vi "Delete_User.vi"(8 "error in (no error)":errorcluster, 11 "Name":string) -> (0 "error out":errorcluster, 3 "Result":bool)   [LabVIEW 2021]
uses:
  <vilib>/regexp/Match Regular Expression.xnode
panel:
  out "concatenated string":string
  out "standard output":string
  out "standard error":string
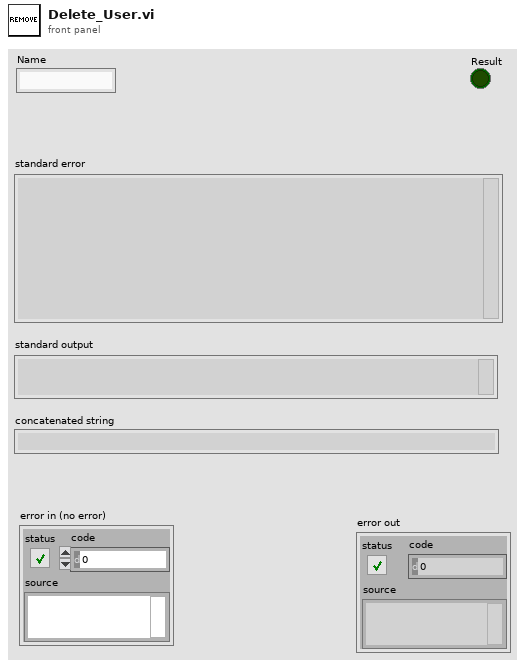
[diagram p1: front panel]
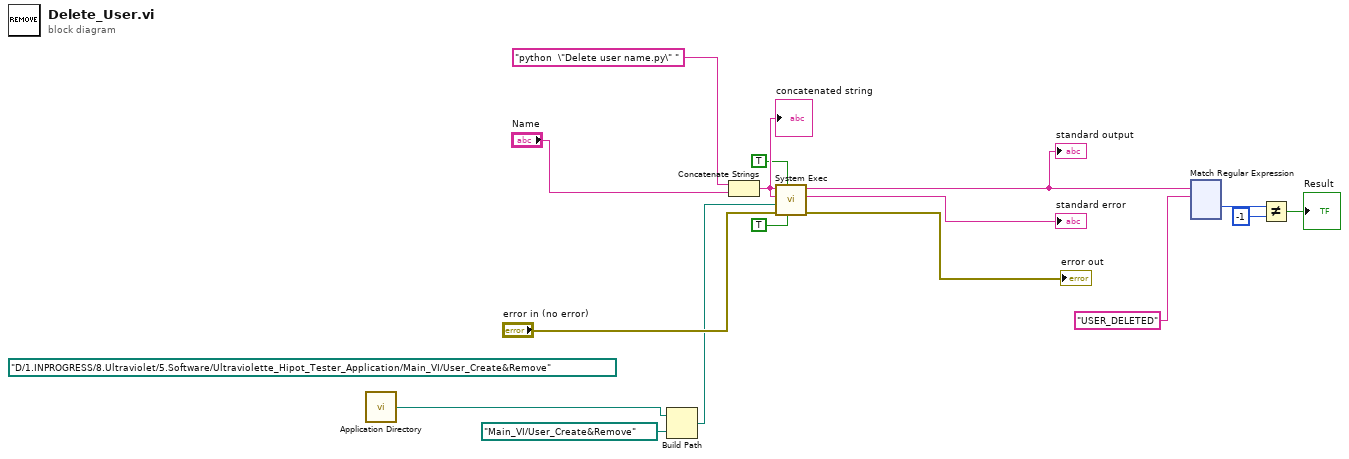
[diagram p0: block diagram]
diagram:
  (unwired) path "D:/1.INPROGRESS/8.Ultraviolet/5.Software/Ultraviolette_Hipot_Tester_Application/Main_VI/User_Create&Remove" ("working directory")
  n1 = call <vilib>:"Application Directory.vi"() -> ("Application Directory"=w2:path)
  n2 = Build Path(base path=w2, name or relative path=path "Main_VI/User_Create&Remove") -> (appended path=w1:path)
  n3 = Concatenate Strings("python  \"Delete user name.py\" " ("command line"), "Name") -> (w14:string)
  "concatenated string" <- w14
  n4 = call <vilib>:"System Exec.vi"("run minimized? (F)"=TRUE, "wait until completion? (T)"=TRUE, "error in (no error)"="error in (no error)", "working directory"=w1, "standard input"=w14, "command line"=w14) -> ("error out"=→"error out":errorcluster, "standard error"=→"standard error":string, "standard output"=w11:string)  [unwired: 2 in, 1 out]
  "standard output" <- w11
  n5 = xnode "Match Regular Expression"("input string"=w11, "regular expression"="USER_DELETED") -> ("offset past match"=w9:i32)  [unwired: 4 in, 4 out]
  n6 = Not Equal?(x=w9, y=-1) -> (x != y?=→"Result":bool)
